vi "VIH HelpGen - Image - Convert Image to 2D Array.vi"(9 "Black & White (F)":bool, 11 "Image Data":T1) -> (0 "columns":i32, 1 "rows":i32, 3 "Image 2D Array":u32[][](array[numeric]) format="%.0x")   [LabVIEW 2014]
doc: "::: VI Helpeks :::\nCopyright (c) 2000-2026 Konstantin Shifershteyn. All rights reserved."
uses:
  <vilib>/picture/picture.llb/imagedata.ctl
panel:
  # "VI Helpeks\nCopyright (c) 2012-2026 Konstantin Shifershteyn"
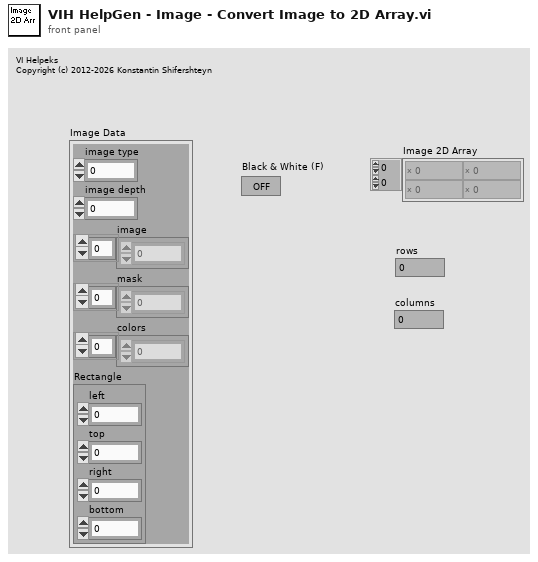
[diagram p1: front panel]
types:
  T1 = typedef "imagedata.ctl" = cluster{"image type":i32, "image depth":i32, "image":u8[], "mask":u8[], "colors":u32[], "Rectangle":cluster{"left":i16, "top":i16, "right":i16, "bottom":i16}}
  T2 = cluster{"left":i16, "top":i16, "right":i16, "bottom":i16}
  T3 = cluster{"left":i32, "top":i32, "right":i32, "bottom":i32}
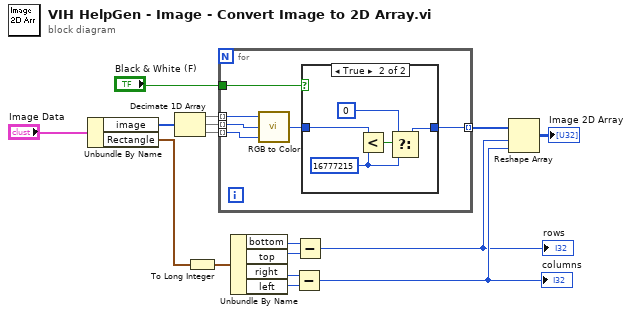
[diagram p0: block diagram]
diagram:
  n1 = Unbundle By Name("Image Data") -> ("image"=w12:u8[], "Rectangle"=w6:T2)
  n2 = Decimate 1D Array(w12) -> (w13:u8[], w14:u8[], w15:u8[])
  n3 = To Long Integer(number=w6) -> (32bit integer=w1:T3)
  n4 = for {
    tunnel: w13 -> [w22] mode=indexing
    tunnel: w14 -> [w21] mode=indexing
    tunnel: w15 -> [w20] mode=indexing
    tunnel: [w19] -> w7 mode=indexing
    tunnel: "Black & White (F)" -> [w17]
    n5 = call <vilib>:"RGB to Color.vi"("B"=w20, "G"=w21, "R"=w22) -> ("Color"=w18:u32)
    n6 = case shown="True" w17 {
      tunnel: [w23 w27] -> w19
      tunnel: w18 -> [w23 w26]
      frame False {
      }
      frame True {
        w24 = u32 16777215
        n7 = Less?(x=w26, y=w24) -> (x < y?=w28:bool)
        n8 = Select(t=u32 0, s=w28, f=w24) -> (s? t:f=w27:u32)
      }
    }
  }
  n9 = Unbundle By Name(w1) -> ("bottom"=w8:i32, "top"=w9:i32, "right"=w10:i32, "left"=w11:i32)
  n10 = Subtract(x=w10, y=w11) -> (x-y=w5:i32)
  "columns" <- w5
  n11 = Subtract(x=w8, y=w9) -> (x-y=w4:i32)
  "rows" <- w4
  n12 = Reshape Array(w7, w4, w5) -> (→"Image 2D Array":u32[][])
